vi "Alarm_Logger.vi"(7 "Alarm Text":string, 8 "error in (no error)":errorcluster, 9 "Alarm Code":i32, 10 "InAlarm":bool, 11 "Log Dir":path) -> (0 "error out":errorcluster)   [LabVIEW 2018]
doc: "Use this template to build a VI to use as a subVI."
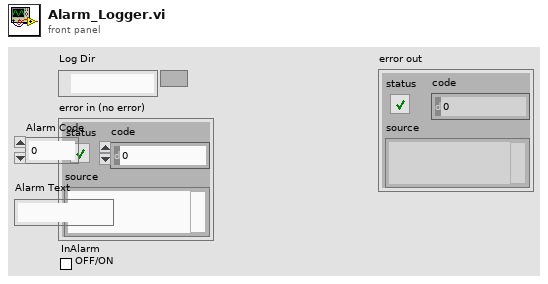
[diagram p1: front panel]
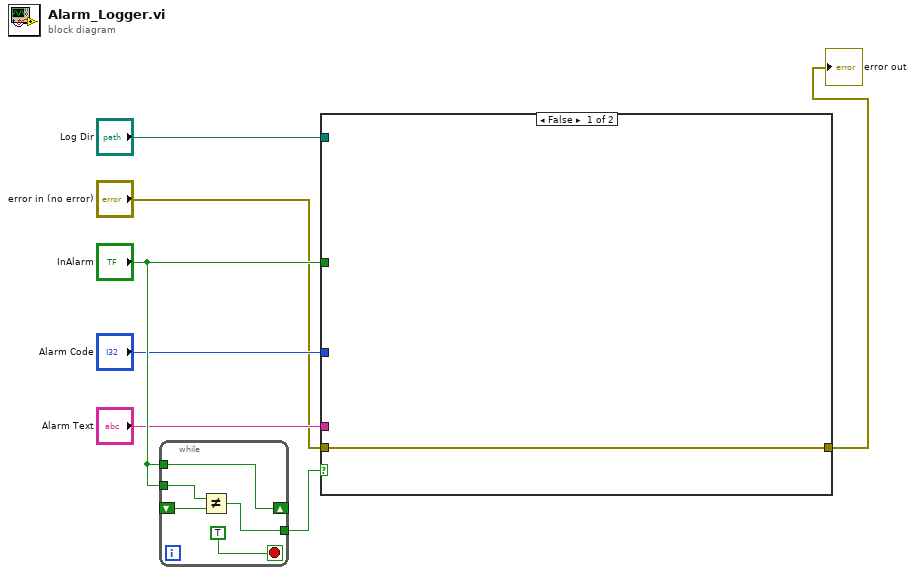
[diagram p0: block diagram]
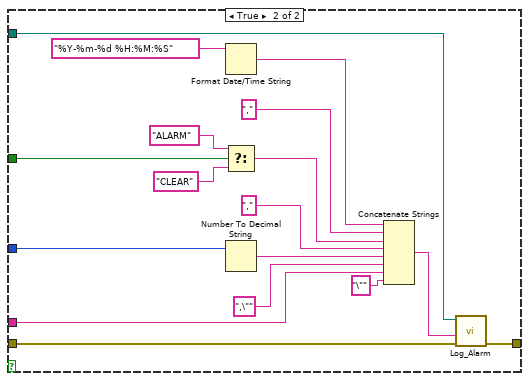
[diagram p2: hidden frame]
diagram:
  n1 = while {
    shift-right: [w10] -> _
    shift-left: _ -> [w11]
    tunnel: "InAlarm" -> [w12]
    tunnel: "InAlarm" -> [w10]
    tunnel: [w8] -> w7
    stop <- TRUE stop-if-true
    n2 = Not Equal?(x=w12, y=w11) -> (x != y?=w8:bool)
  }
  n3 = case shown="False" w7 {
    tunnel: "InAlarm" -> [_ w30]
    tunnel: "Alarm Code" -> [_ w26]
    tunnel: "Alarm Text" -> [_ w19]
    tunnel: "Log Dir" -> [_ w16]
    tunnel: "error in (no error)" -> [w13 w15]
    tunnel: [w13 w14] -> w1
    frame False {
    }
    frame True {
      n4 = Format Date/Time String(time format string (%c)="%Y-%m-%d %H:%M:%S") -> (date/time string=w25:string)  [unwired: 2 in]
      n5 = Select(t="ALARM", s=w30, f="CLEAR") -> (s? t:f=w23:string)
      n6 = Number To Decimal String(number=w26) -> (decimal integer string=w21:string)  [unwired: 1 in]
      n7 = Concatenate Strings(w25, ",", w23, ",", w21, ",\"", w19, "\"") -> (w17:string)
      n8 = call "Log_Alarm.vi"("error in (no error)"=w15, "Line"=w17, "Log Dir"=w16) -> ("error out"=w14:errorcluster)  [unwired: 8 in]
    }
  }
  "error out" <- w1
